vi "Update Context for Owned Processes.vi"(8 "error in (no error)":errorcluster, 11 "Application In":refnum<class "Application.lvclass">) -> (0 "error out":errorcluster, 3 "Application Out":refnum<class "Application.lvclass">)   [LabVIEW 2020, in "Application.lvclass"]
uses:
  Application.lvclass
  C:/git/astemes-triarc-framework/source/Framework/Process/Process.lvclass
  Application.lvclass/Application.ctl
  Process/Process.lvclass/Process.ctl
  Process/Public/Lifecycle/Get Lifecycle State.vi
  <vilib>/Utility/error.llb/Clear Errors.vi
  <vilib>/Utility/error.llb/Error Cluster From Error Code.vi
  Process/Process.lvclass
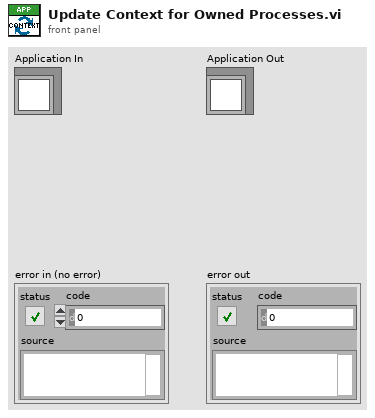
[diagram p1: front panel]
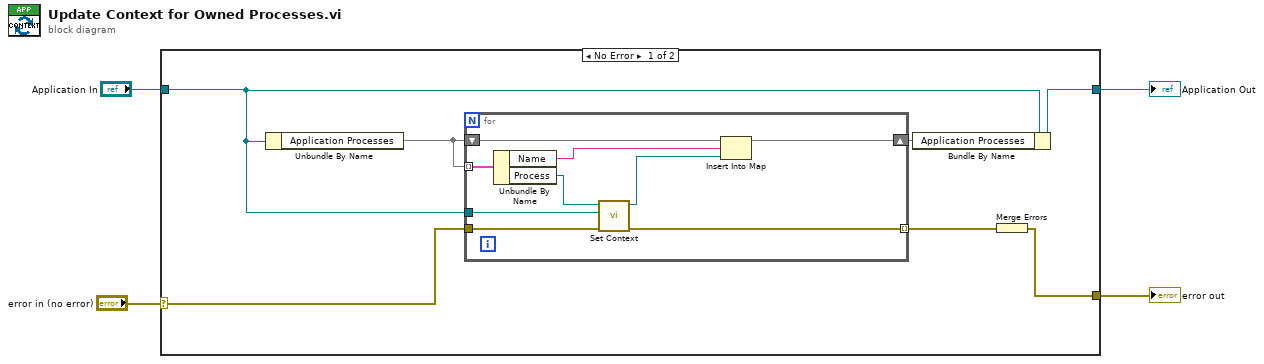
[diagram p0: block diagram]
diagram:
  n1 = case shown="No Error" "error in (no error)" {
    selector: "error in (no error)" -> [w8 w21]
    tunnel: [w11 w22] -> w4
    tunnel: [w10 w21] -> w3
    tunnel: "Application In" -> [w5 w22]
    frame No Error {
      n2 = Unbundle By Name(w5) -> ("Application Processes"=w7:map{string, refnum<class "Process.lvclass">})
      n3 = for {
        tunnel: w8 -> [w20]
        tunnel: w5 -> [w19]
        tunnel: [w13] -> w9 mode=indexing
        tunnel: w7 -> [w18] mode=indexing
        shift-right: [w14] -> w6
        shift-left: w7 -> [w16]
        n4 = Unbundle By Name(w18) -> ("Name"=w15:string, "Process"=w17:refnum<class "Process.lvclass">)
        n5 = call "Set Context.vi"("error in (no error)"=w20, "Process Context"=w19, "Process In"=w17) -> ("error out"=w13:errorcluster, "Process Out"=w12:refnum<class "Process.lvclass">)  [unwired: 7 in]
        n6 = Insert Into Map(map in=w16, key=w15, value=w12) -> (map out=w14:map{string, refnum<class "Process.lvclass">})  [unwired: 2 out]
      }
      n7 = Bundle By Name(cluster=w5, "Application Processes"=w6) -> (w11:refnum<class "Application.lvclass">)
      n8 = Merge Errors(w9) -> (w10:errorcluster)
    }
    frame Error {
    }
  }
  "Application Out" <- w4
  "error out" <- w3
